vi "DAC Configure.vi"(8 "error in":errorcluster, 11 "DAC Vacum Pressure in":refnum<class "DAC Vacum Pressure.lvclass">) -> (0 "error out":errorcluster, 3 "DAC Vacum Pressure out":refnum<class "DAC Vacum Pressure.lvclass">)   [LabVIEW 2019, in "DAC.lvlib" / "DAC Vacum Pressure.lvclass"]
uses:
  DAC Vacum Pressure.lvclass
  DAC.lvclass
  <vilib>/DAQmx/create/channels.llb/DAQmx Create Channel (AI-Current-Basic).vi
  <resource>/objmgr/daqmx.rc
  C:/Users/wg/Documents/LV_Projects/test-stand/App/DAC/DAC.lvclass
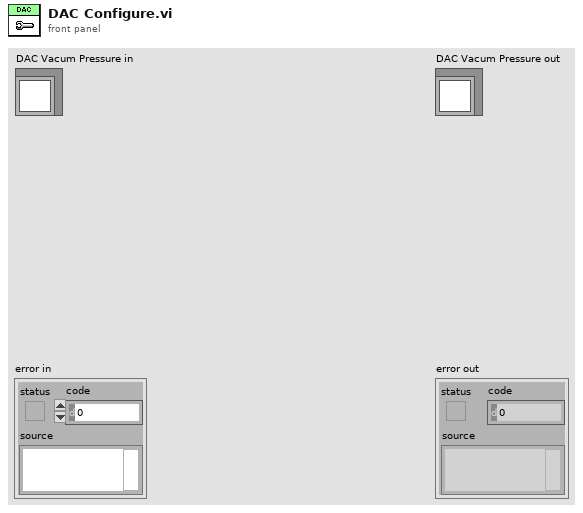
[diagram p1: front panel]
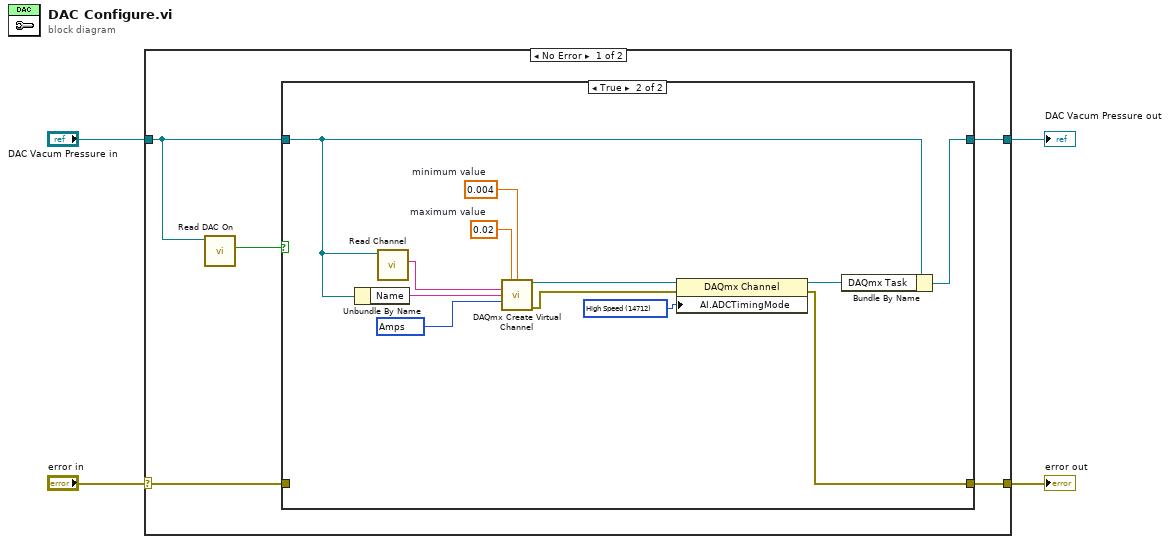
[diagram p0: block diagram]
diagram:
  n1 = case shown="No Error" "error in" {
    selector: "error in" -> [w6 w25]
    tunnel: [w5 w25] -> w4
    tunnel: [w7 w24] -> w3
    tunnel: "DAC Vacum Pressure in" -> [w9 w24]
    frame No Error {
      n2 = call "Read DAC On.vi"("DAC in"=w9) -> ("DAC On"=w8:bool)  [unwired: 8 in, 2 out]
      n3 = case shown="True" w8 {
        tunnel: w9 -> [w11 w14]
        tunnel: [w11 w23] -> w7
        tunnel: w6 -> [w10 _]
        tunnel: [w10 w16] -> w5
        frame False {
          # "Temperature measurement is off."
        }
        frame True {
          w12 = 0.02  # maximum value
          w13 = 0.004  # minimum value
          w18 = 14712 items=["Automatic"=16097, "High Resolution"=10195, "High Speed"=14712, "Best 50 Hz Rejection"=14713, "Best 60 Hz Rejection"=14714, "Custom"=10137] ("AI.ADCTimingMode")
          w21 = 10342 items=["Amps"=10342, "From Custom Scale"=10065] ("units")
          # "Temperature measurement is on."
          n4 = Unbundle By Name(w14) -> ("Name"=w22:string)
          n5 = call "Read Channel.vi"("DAC in"=w14) -> ("Channel"=w15:string)  [unwired: 8 in, 2 out]
          n6 = call-poly <vilib>:"DAQmx Create Virtual Channel.vi"("maximum value"=w12, "minimum value"=w13, "physical channels"=w15, "name to assign"=w22, "units"=w21) -> ("task out"=w20:refnum<k21>, "error out"=w17:errorcluster)  [unwired: 9 in]
          n7 = property class="DAQmx Channel"(reference=w20, error in=w17, "AI.ADCTimingMode"=w18) -> (reference out=w19:refnum<k21>, error out=w16:errorcluster)
          n8 = Bundle By Name(cluster=w14, "DAQmx Task"=w19) -> (w23:refnum<class "DAC Vacum Pressure.lvclass">)
        }
      }
    }
    frame Error {
    }
  }
  "error out" <- w4
  "DAC Vacum Pressure out" <- w3
